vi "Get Matrix of DBL.vi"(8 "error in (no error)":errorcluster, 10 "Name":string, 11 "json class in":refnum<class "json class.lvclass">) -> (0 "error out":errorcluster, 2 "Array":dbl[][](array[numeric]), 3 "json class out":refnum<class "json class.lvclass">)   [LabVIEW 2021, in "Config Library.lvlib" / "json class.lvclass"]
uses:
  json class.lvclass
  json class.lvclass/json class.ctl
  <vilib>/addons/JSON API/JSON Array/JSON Array.lvclass
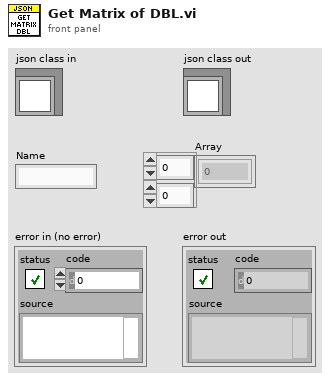
[diagram p1: front panel]
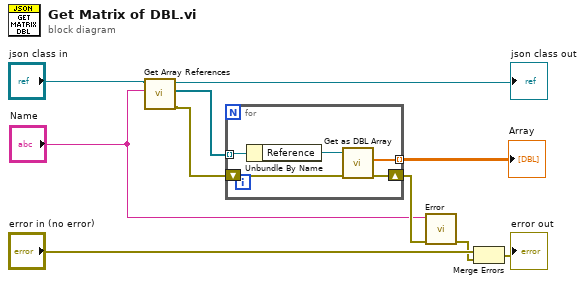
[diagram p0: block diagram]
diagram:
  n1 = call "Get Array References.vi"("Name"="Name", "json class in"="json class in") -> ("error out"=w6:errorcluster, "Array json class"=w7:refnum<class "json class.lvclass">[], "json class out"=→"json class out":refnum<class "json class.lvclass">)  [unwired: 7 in]
  n2 = for {
    tunnel: w7 -> [w15] mode=indexing
    tunnel: [w12] -> w5 mode=indexing
    shift-right: [w11] -> w4
    shift-left: w6 -> [w13]
    n3 = Unbundle By Name(w15) -> ("Reference"=w14:refnum<class "JSON Value.lvclass">)
    n4 = call <vilib>:"Get as DBL Array.vi"("error in (no error)"=w13, "JSON Array in"=w14) -> ("error out"=w11:errorcluster, "Array of numbers"=w12:dbl[])  [unwired: 7 in, 1 out]
  }
  "Array" <- w5
  n5 = call "Error.vi"("error in (no error)"=w4, "Name"="Name") -> ("error out"=w1:errorcluster)  [unwired: 9 in]
  n6 = Merge Errors("error in (no error)", w1) -> (→"error out":errorcluster)
